vi "Connect_direct.vi"   [LabVIEW 2020, in "ORM_API_jdp.lvlib"]
uses:
  ORM_API_jdp.lvlib
  <vilib>/Viviota/shared/ORM_pgsql_jdp.lvlibp/dbc/DBC.lvclass
  <vilib>/Viviota/shared/ORM_sqlite_jdp.lvlibp/dbc/DBC.lvclass
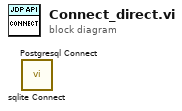
[diagram p0: block diagram]
diagram:
  n1 = call <vilib>:"sqlite Connect.vi"() -> ()  [unwired: 10 in, 2 out]
  n2 = call <vilib>:"Postgresql Connect.vi"() -> ()  [unwired: 10 in, 2 out]
